vi "WebDAV_GetNew.vi"(6 "IP myRIO":string="172.22.11.2", 8 "error in (no error)":errorcluster, 9 "user":string, 10 "password":string, 11 "local file path":path) -> (0 "error out":errorcluster, 3 "dowloads":string[](array[string]))   [LabVIEW 2025]
uses:
  <vilib>/WebDAVClient/NI_WebDAV.lvlib
  <vilib>/WebDAVClient/Advanced/Get File.vi
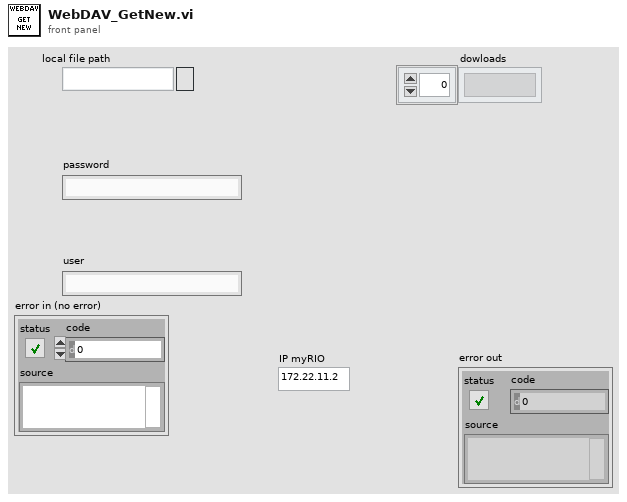
[diagram p1: front panel]
types:
  T1 = typedef "NI_WebDAV.lvlib/SessionHandle.ctl" = refnum<k1>
  T2 = typedef "NI_WebDAV.lvlib/FileInfo.ctl" = cluster{"type":string, "size":u64, "last modification":timestamp, "display name":string, "uri":string}
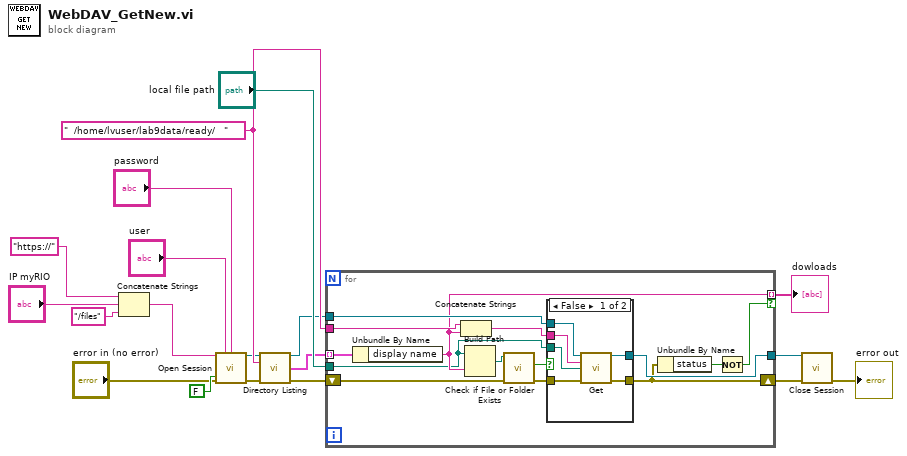
[diagram p0: block diagram]
diagram:
  w14 = "  /home/lvuser/lab9data/ready/   " ("relative uri")
  n1 = Concatenate Strings("https://" ("string"), "IP myRIO", "/files" ("string")) -> (w10:string)
  n2 = call <vilib>:"Open Session.vi"("host uri prefix"=w10, "username"="user", "password"="password", "error in (no error)"="error in (no error)", "verify server?"=FALSE) -> ("session handle out"=w9:T1, "error out"=w8:errorcluster)  [unwired: 9 in]
  n3 = call <vilib>:"Directory Listing.vi"("session handle"=w9, "relative uri"=w14, "error in (no error)"=w8) -> ("session handle out"=w13:T1, "file list"=w11:T2[], "error out"=w12:errorcluster)  [unwired: 9 in, 1 out]
  n4 = for {
    tunnel: w11 -> [w33] mode=indexing
    shift-right: [w24] -> w18
    shift-left: w12 -> [w26]
    tunnel: w13 -> [w32]
    tunnel: w14 -> [w29]
    tunnel: [w21] -> w15 mode=indexing if=w23
    tunnel: "local file path" -> [w20]
    tunnel: [w30] -> w17
    n5 = Unbundle By Name(w33) -> ("display name"=w21:string)
    n6 = Concatenate Strings(w29, w21) -> (w31:string)
    n7 = Build Path(base path=w20, name or relative path=w21) -> (appended path=w28:path)
    n8 = call <vilib>:"Check if File or Folder Exists.vi"("error in (no error)"=w26, "path"=w28) -> ("error out"=w25:errorcluster, "file or folder exists?"=w27:bool)  [unwired: 7 in, 1 out]
    n9 = case shown="False" w27 {
      tunnel: w32 -> [w39 w40]
      tunnel: w20 -> [w38 _]
      tunnel: w25 -> [w37 w41]
      tunnel: w31 -> [w34 _]
      tunnel: [w35 w40] -> w30
      tunnel: [w36 w41] -> w24
      frame False {
        n10 = call-poly <vilib>:"Get.vi"("session handle"=w39, "relative uri"=w34, "local file path"=w38, "error in (no error)"=w37) -> ("session handle out"=w35:T1, "error out"=w36:errorcluster)  [unwired: 9 in, 1 out]
      }
      frame True {
      }
    }
    n11 = Unbundle By Name(w24) -> ("status"=w22:bool)
    n12 = Not(x=w22) -> (.not. x?=w23:bool)
  }
  "dowloads" <- w15
  n13 = call <vilib>:"Close Session.vi"("session handle"=w17, "error in (no error)"=w18) -> ("error out"=→"error out":errorcluster)  [unwired: 13 in]
